vi "DAQ config DAQmx config (AO and AI).vi"(8 "error in (no error)":errorcluster, 10 "AO Config":T13, 11 "AI Config":T8) -> (0 "error out":errorcluster, 2 "AO config":T1 {"output terminal configuration" items=[""=-1, "Differential"=10106, "Pseudodifferential"=12529]}, 3 "AI config":T4 {"input terminal configuration" items=[""=-1, "Differential"=10106, "Pseudodifferential"=12529]; "Coupling" items=["AC"=10045, "DC"=10050, "GND"=10066]})   [LabVIEW 2019, in "Instrument.Lockin.lvlib" / "Instrument.DAQ.lvclass"]
uses:
  Instrument.DAQ.lvclass
  Lockin.Typedefs/DAQ/DAQ.Config.AO--Cluster--Array.ctl
  Lockin.Typedefs/DAQ/DAQ.Config.AO--Cluster.ctl
  Lockin.Typedefs/DAQ/DAQ.Config.AO.Range--enum.ctl
  Lockin.Typedefs/DAQ/DAQ.TerminalConfiguration--enum.ctl
  Lockin.Typedefs/DAQ/DAQ.Config.AI--Cluster--Array.ctl
  Lockin.Typedefs/DAQ/DAQ.Config.AI--Cluster.ctl
  Lockin.Typedefs/DAQ/DAQ.Config.AI.Coupling--enum.ctl
  Lockin.Typedefs/DAQ/DAQ.Config.AI.Range--enum.ctl
  DAQmx/typedefs/DAQmx.Config.AO.Range--enum.ctl
  DAQmx/DAQmx.lvclass
  DAQmx/typedefs/DAQmx.Config.AO--Cluster.ctl
  DAQmx/typedefs/DAQmx.Config.AI.Coupling--enum.ctl
  DAQmx/typedefs/DAQmx.Config.AI.Range--enum.ctl
  DAQmx/typedefs/DAQmx.Config.AI--Cluster.ctl
  DAQmx/typedefs/DAQmx.Config.AO--Cluster--Array.ctl
  DAQmx/typedefs/DAQmx.Config.AI--Cluster--Array.ctl
  Lockin.Typedefs/Lockin.Typedefs.lvlib
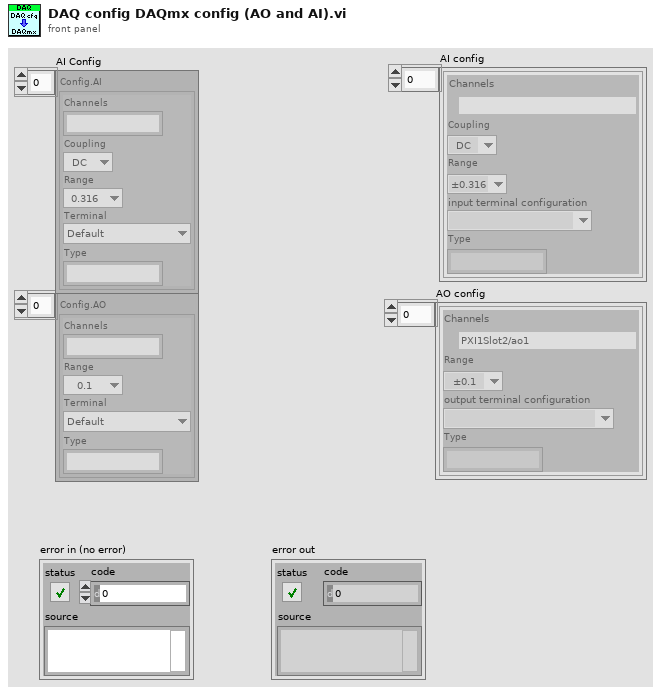
[diagram p1: front panel]
types:
  T1 = typedef "DAQmx.lvclass/DAQmx.Config.AO--Cluster--Array.ctl" = T2[]
  T2 = typedef "DAQmx.lvclass/DAQmx.Config.AO--Cluster.ctl" = cluster{"Channels":tag, "Range":T3, "output terminal configuration":i32, "Type":string}
  T3 = typedef "DAQmx.lvclass/DAQmx.Config.AO.Range--enum.ctl" = enum16{"±0.1", "±1.0", "±3.5", "±10.0"}
  T4 = typedef "DAQmx.lvclass/DAQmx.Config.AI--Cluster--Array.ctl" = T5[]
  T5 = typedef "DAQmx.lvclass/DAQmx.Config.AI--Cluster.ctl" = cluster{"Channels":tag, "Coupling":T6, "Range":T7, "input terminal configuration":i32, "Type":string}
  T6 = typedef "DAQmx.lvclass/DAQmx.Config.AI.Coupling--enum.ctl" = u16
  T7 = typedef "DAQmx.lvclass/DAQmx.Config.AI.Range--enum.ctl" = enum16{"±0.316", "±1.00", "±3.16", "±10.0", "±31.6", "±42.4"}
  T8 = typedef "Lockin.Typedefs.lvlib/DAQ.Config.AI--Cluster--Array.ctl" = T9[]
  T9 = typedef "Lockin.Typedefs.lvlib/DAQ.Config.AI--Cluster.ctl" = cluster{"Channels":string, "Coupling":T10, "Range":T11, "Terminal":T12, "Type":string}
  T10 = typedef "Lockin.Typedefs.lvlib/DAQ.Config.AI.Coupling--enum.ctl" = enum16{"AC", "DC", "GND", ""}
  T11 = typedef "Lockin.Typedefs.lvlib/DAQ.Config.AI.Range--enum.ctl" = enum16{"0.316", "1.00", "3.16", "10.0", "31.6", "42.4", ""}
  T12 = typedef "Lockin.Typedefs.lvlib/DAQ.TerminalConfiguration--enum.ctl" = enum16{"Default", "Differential", "Pseudodifferential", ""}
  T13 = typedef "Lockin.Typedefs.lvlib/DAQ.Config.AO--Cluster--Array.ctl" = T14[]
  T14 = typedef "Lockin.Typedefs.lvlib/DAQ.Config.AO--Cluster.ctl" = cluster{"Channels":string, "Range":T15, "Terminal":T12, "Type":string}
  T15 = typedef "Lockin.Typedefs.lvlib/DAQ.Config.AO.Range--enum.ctl" = enum16{"0.1", "1.0", "3.5", "10.0", ""}
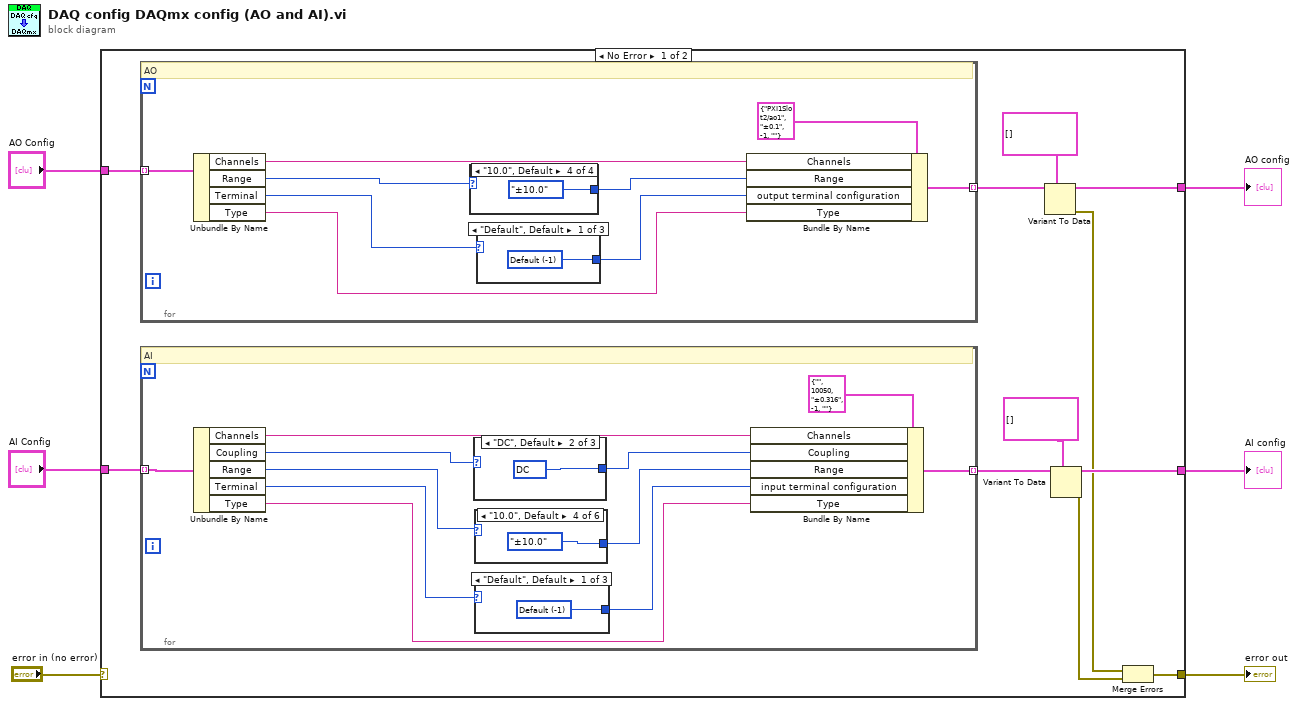
[diagram p0: block diagram]
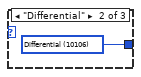
[diagram p2: hidden frame]
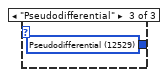
[diagram p3: hidden frame]
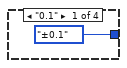
[diagram p4: hidden frame]
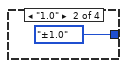
[diagram p5: hidden frame]
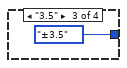
[diagram p6: hidden frame]
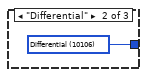
[diagram p7: hidden frame]
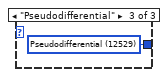
[diagram p8: hidden frame]
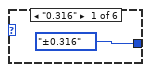
[diagram p9: hidden frame]
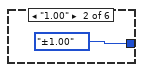
[diagram p10: hidden frame]
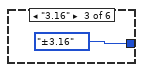
[diagram p11: hidden frame]
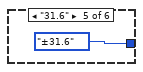
[diagram p12: hidden frame]
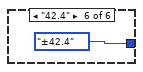
[diagram p13: hidden frame]
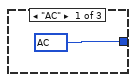
[diagram p14: hidden frame]
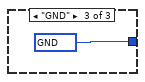
[diagram p15: hidden frame]
diagram:
  n1 = case shown="No Error" "error in (no error)" {
    selector: "error in (no error)" -> [_ w57]
    tunnel: "AO Config" -> [w16 _]
    tunnel: [w7 w57] -> w4
    tunnel: "AI Config" -> [w17 _]
    tunnel: [w13 _] -> w2
    tunnel: [w12 _] -> w1
    frame No Error {
      n2 = for {
        tunnel: w16 -> [w26] mode=indexing
        tunnel: [w25] -> w14 mode=indexing
        # "AO"
        n3 = Unbundle By Name(w26) -> ("Channels"=w23:string, "Range"=w21:T15, "Terminal"=w20:T12, "Type"=w18:string)
        n4 = case shown="\"10.0\", Default" w21 {
          tunnel: [DAQmx.Config.AO.Range--enum."±0.1" ("Range") DAQmx.Config.AO.Range--enum."±1.0" ("Range") DAQmx.Config.AO.Range--enum."±3.5" ("Range") DAQmx.Config.AO.Range--enum."±10.0" ("Range")] -> w22
          frame "0.1" {
          }
          frame "1.0" {
          }
          frame "3.5" {
          }
          frame "10.0", Default {
          }
        }
        n5 = case shown="\"Default\", Default" w20 {
          tunnel: [w27 w28 w29] -> w19
          frame "Default", Default {
            w27 = -1 items=["Default"=-1, "Differential"=10106, "Pseudodifferential"=12529] ("output terminal configuration")
          }
          frame "Differential" {
            w28 = 10106 items=["Default"=-1, "Differential"=10106, "Pseudodifferential"=12529] ("output terminal configuration")
          }
          frame "Pseudodifferential" {
            w29 = 12529 items=["Default"=-1, "Differential"=10106, "Pseudodifferential"=12529] ("output terminal configuration")
          }
        }
        n6 = Bundle By Name(cluster=T2 {"Channels"="PXI1Slot2/ao1", "Range"=enum."±0.1", "output terminal configuration"=-1, "Type"=""} ("Config.AO"), "Channels"=w23, "Range"=w22, "output terminal configuration"=w19, "Type"=w18) -> (w25:T2)
      }
      n7 = for {
        tunnel: [w44] -> w15 mode=indexing
        tunnel: w17 -> [w43] mode=indexing
        # "AI"
        n8 = Unbundle By Name(w43) -> ("Channels"=w42:string, "Coupling"=w40:T10, "Range"=w38:T11, "Terminal"=w37:T12, "Type"=w34:string)
        n9 = case shown="\"DC\", Default" w40 {
          tunnel: [w54 w55 w56] -> w39
          frame "AC" {
            w54 = T6 10045 items=["AC"=10045, "DC"=10050, "GND"=10066] ("Coupling")
          }
          frame "DC", Default {
            w55 = T6 10050 items=["AC"=10045, "DC"=10050, "GND"=10066] ("Coupling")
          }
          frame "GND" {
            w56 = T6 10066 items=["AC"=10045, "DC"=10050, "GND"=10066] ("Coupling")
          }
        }
        n10 = case shown="\"10.0\", Default" w38 {
          tunnel: [DAQmx.Config.AI.Range--enum."±0.316" ("Range") DAQmx.Config.AI.Range--enum."±1.00" ("Range") DAQmx.Config.AI.Range--enum."±3.16" ("Range") DAQmx.Config.AI.Range--enum."±10.0" ("Range") DAQmx.Config.AI.Range--enum."±31.6" ("Range") DAQmx.Config.AI.Range--enum."±42.4" ("Range")] -> w36
          frame "0.316" {
          }
          frame "1.00" {
          }
          frame "3.16" {
          }
          frame "10.0", Default {
          }
          frame "31.6" {
          }
          frame "42.4" {
          }
        }
        n11 = case shown="\"Default\", Default" w37 {
          tunnel: [w45 w46 w47] -> w35
          frame "Default", Default {
            w45 = -1 items=["Default"=-1, "Differential"=10106, "Pseudodifferential"=12529] ("output terminal configuration")
          }
          frame "Differential" {
            w46 = 10106 items=["Default"=-1, "Differential"=10106, "Pseudodifferential"=12529] ("output terminal configuration")
          }
          frame "Pseudodifferential" {
            w47 = 12529 items=["Default"=-1, "Differential"=10106, "Pseudodifferential"=12529] ("output terminal configuration")
          }
        }
        n12 = Bundle By Name(cluster=T5 {"Channels"="", "Coupling"=10050, "Range"=enum."±0.316", "input terminal configuration"=-1, "Type"=""} ("Config.AI"), "Channels"=w42, "Coupling"=w39, "Range"=w36, "input terminal configuration"=w35, "Type"=w34) -> (w44:T5)
      }
      n13 = Variant To Data(type=T1 [] ("AOconfig"), Variant=w14) -> (data=w12:T1, error out=w9:errorcluster)  [unwired: 1 in]
      n14 = Variant To Data(type=T4 [] ("AIconfig"), Variant=w15) -> (data=w13:T4, error out=w8:errorcluster)  [unwired: 1 in]
      n15 = Merge Errors(w9, w8) -> (w7:errorcluster)
    }
    frame Error {
    }
  }
  "error out" <- w4
  "AI config" <- w2
  "AO config" <- w1
